vi "Generate Support files File paths.vi"(4 "error in":errorcluster, 6 "base path":path, 7 "ProjectName":T1) -> (0 "error out":errorcluster, 1 "Log path":path, 2 ".ini path":path)   [LabVIEW 2013]
doc: "This .vi generates the filepaths to the various support files and stores that in a global."
uses:
  Config/ProjectName enum.ctl
  Config/User interface config file selector enum.ctl
  Config/Config file functional global mode enum.ctl
  FileIO lib.lvlib
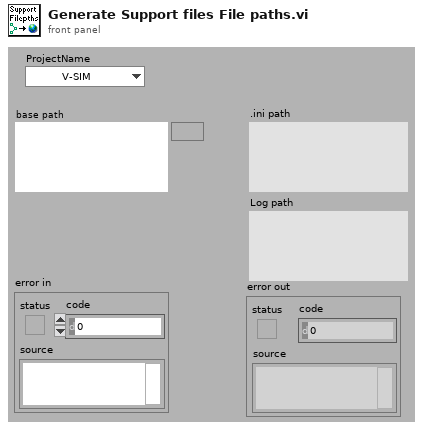
[diagram p1: front panel]
types:
  T1 = typedef "ProjectName enum.ctl" = enum16{"V-SIM", "SPIM", "TEMca2", "undefined", "HHMI Panels", "Wing Beat Analyzer"}
  T2 = typedef "User interface config file selector enum.ctl" = enum16{"MAIN"}
  T3 = typedef "Config file functional global mode enum.ctl" = enum16{"Set Filepath", "Read file", "Rewrite file"}
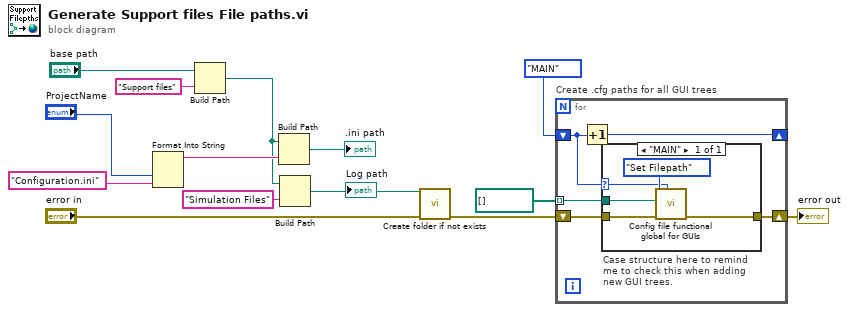
[diagram p0: block diagram]
diagram:
  n1 = Format Into String("ProjectName", "Configuration.ini" ("name or relative path")) -> (resulting string=w11:string)  [unwired: 3 in, 1 out]
  n2 = Build Path(base path="base path", name or relative path="Support files" ("string")) -> (appended path=w6:path)
  n3 = Build Path(base path=w6, name or relative path=w11) -> (appended path=→".ini path":path)
  n4 = Build Path(base path=w6, name or relative path="Simulation Files") -> (appended path=w3:path)
  "Log path" <- w3
  n5 = call "Create folder if not exists.vi"("error in"="error in", "Path in"=w3) -> ("error out"=w1:errorcluster)  [unwired: 7 in, 2 out]
  n6 = for "Create .cfg paths for all GUI trees" {
    tunnel: path[] [] -> [w18] mode=indexing
    shift-right: [w17] -> w14
    shift-left: w1 -> [w19]
    shift-right: [w16] -> _
    shift-left: User_interface_config_file_selector_enum."MAIN" ("Config file") -> [w15]
    # "Case structure here to remind\nme to check this when adding\nnew GUI trees."
    n7 = Increment(x=w15) -> (x+1=w16:T2)
    n8 = case shown="\"MAIN\"" w15 {
      selector: w15 -> [w20]
      tunnel: w19 -> [w23]
      tunnel: w18 -> [w22]
      tunnel: [w21] -> w17
      frame "MAIN" {
        n9 = call "Config file functional global for GUIs.vi"("GUI elements"=w20, "error in"=w23, "file path"=w22, "Mode"=Config_file_functional_global_mode_enum."Set Filepath") -> ("error out"=w21:errorcluster)  [unwired: 1 in, 6 out]
      }
    }
  }
  "error out" <- w14
